vi "SMS Analysis Interface User Get Data Path.vi"() -> (4 "Transfer Log Path":string, 6 "Image Name":string, 8 "Frames":u32, 10 "Cycles":u16, 13 "setupName":string, 14 "channelCode":u8, 15 "Error":errorcluster)   [LabVIEW 2016]
uses:
  Tools/Metadata/Microscope Metadata/Device Metadata Types/Capture Metadata.ctl
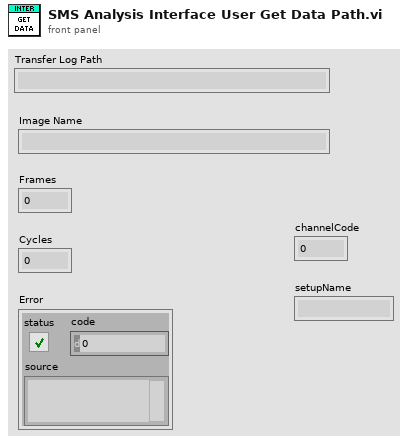
[diagram p1: front panel]
types:
  T1 = typedef "Capture Metadata.ctl" = cluster{"Capture_Exposure_sec":dbl, "Cycles":u16, "Frames":u32, "No_of_Z_Steps":u16, "Z_Step_Size_um":dbl, "Init_Z_Position_um":dbl, "Save_Path":string, "Line_Scan":bool, "Line_Scan_Mode":string, "channelCode":u8, "setupName":string}
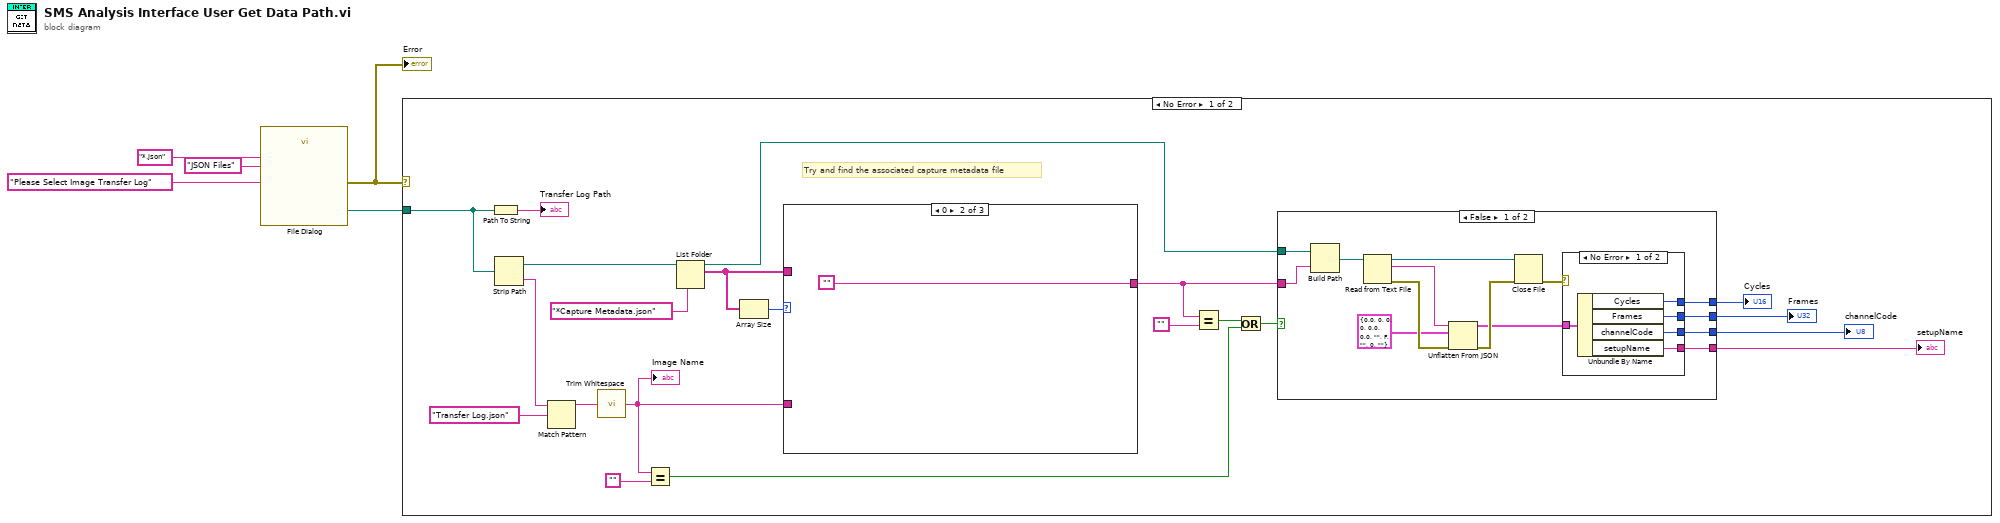
[diagram p0: block diagram]
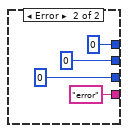
[diagram p2: hidden frame]
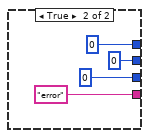
[diagram p3: hidden frame]
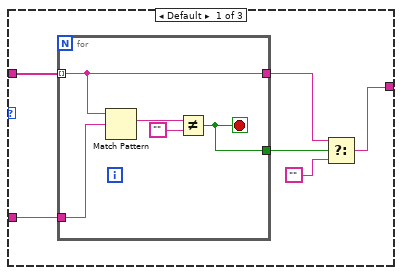
[diagram p4: hidden frame]
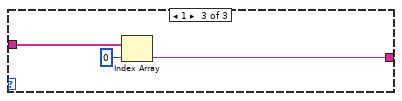
[diagram p5: hidden frame]
diagram:
  n1 = call "File Dialog"("prompt"="Please Select Image Transfer Log", "pattern (all files)"="*.json", "pattern label"="JSON Files") -> ("selected path"=w2:path, "error out"=w1:errorcluster)  [unwired: 9 in, 2 out]
  "Error" <- w1
  n2 = case shown="No Error" w1 {
    tunnel: w2 -> [w25 _]
    frame No Error {
      # "Try and find the associated capture metadata file"
      n3 = Path To String(path=w25) -> (string=→"Transfer Log Path":string)
      n4 = Strip Path(path=w25) -> (stripped path=w24:path, name=w21:string)
      n5 = Match Pattern(string=w21, regular expression="Transfer Log.json") -> (before substring=w20:string)  [unwired: 1 in, 3 out]
      n6 = call <vilib>:"Trim Whitespace.vi"("string"=w20) -> ("trimmed string"=w17:string)  [unwired: 1 in]
      "Image Name" <- w17
      n7 = Equal?(x=w17, y="") -> (x = y?=w13:bool)
      n8 = List Folder(path=w24, pattern="*Capture Metadata.json") -> (path out=w10:path, filenames=w18:string[])  [unwired: 2 in, 2 out]
      n9 = Array Size(array=w18) -> (size(s)=w19:i32)
      n10 = case shown="0" w19 {
        tunnel: w18 -> [w59 _ w68]
        tunnel: [w54 "" w66] -> w11
        tunnel: w17 -> [w58 _ _]
        frame Default {
          n11 = for {
            tunnel: w59 -> [w61] mode=indexing
            tunnel: w58 -> [w64]
            tunnel: [w61] -> w56
            tunnel: [w60] -> w57
            stop <- w60 stop-if-true
            n12 = Match Pattern(string=w61, regular expression=w64) -> (match substring=w62:string)  [unwired: 1 in, 3 out]
            n13 = Not Equal?(x=w62, y="") -> (x != y?=w60:bool)
          }
          n14 = Select(t=w56, s=w57, f="") -> (s? t:f=w54:string)
        }
        frame 0 {
        }
        frame 1 {
          n15 = Index Array(array=w68, index=0) -> (element=w66:string)
        }
      }
      n16 = Equal?(x=w11, y="") -> (x = y?=w14:bool)
      n17 = Or(x=w14, y=w13) -> (x .or. y?=w12:bool)
      n18 = case shown="False" w12 {
        tunnel: w11 -> [w39 _]
        tunnel: w10 -> [w40 _]
        tunnel: [w30 u16 0 ("Cycles")] -> w9
        tunnel: [w29 u32 0 ("Frames")] -> w8
        tunnel: [w28 u8 0 ("channelCode")] -> w7
        tunnel: [w27 "error" ("setupName")] -> w6
        frame False {
          n19 = Build Path(base path=w40, name or relative path=w39) -> (appended path=w38:path)
          n20 = Read from Text File(file (use dialog)=w38) -> (refnum out=w37:refnum<file>, text=w36:string, error out=w35:errorcluster)  [unwired: 3 in, 1 out]
          n21 = Unflatten From JSON(JSON string=w36, type and defaults=T1 {"Capture_Exposure_sec"=0.0, "Cycles"=0, "Frames"=0, "No_of_Z_Steps"=0, "Z_Step_Size_um"=0.0, "Init_Z_Position_um"=0.0, "Save_Path"="", "Line_Scan"=FALSE, "Line_Scan_Mode"="", "channelCode"=0, "setupName"=""} ("Capture Metadata"), error in (no error)=w35) -> (value=w31:T1, error out=w34:errorcluster)  [unwired: 4 in]
          n22 = Close File(refnum=w37, error in=w34) -> (error out=w32:errorcluster)  [unwired: 1 out]
          n23 = case shown="No Error" w32 {
            tunnel: w31 -> [w45 _]
            tunnel: [w44 u16 0 ("Cycles")] -> w30
            tunnel: [w43 u32 0 ("Frames")] -> w29
            tunnel: [w42 u8 0 ("channelCode")] -> w28
            tunnel: [w41 "error" ("setupName")] -> w27
            frame No Error {
              n24 = Unbundle By Name(w45) -> ("Cycles"=w44:u16, "Frames"=w43:u32, "channelCode"=w42:u8, "setupName"=w41:string)
            }
            frame Error {
            }
          }
        }
        frame True {
        }
      }
      "Cycles" <- w9
      "Frames" <- w8
      "channelCode" <- w7
      "setupName" <- w6
    }
    frame Error {
    }
  }
